vi "Get Target Branch Names.vi"(8 "error in":errorcluster, 11 "Peer Review in":refnum<class "Peer Review.lvclass">) -> (0 "error out":errorcluster, 3 "Peer Review out":refnum<class "Peer Review.lvclass">)   [LabVIEW 2020, in "Peer Review.lvclass"]
uses:
  Peer Review.lvclass
  Peer Review.lvclass/Peer Review.ctl
  <vilib>/Utility/error.llb/Trim Whitespace One-Sided.vi
  <vilib>/regexp/Match Regular Expression.xnode
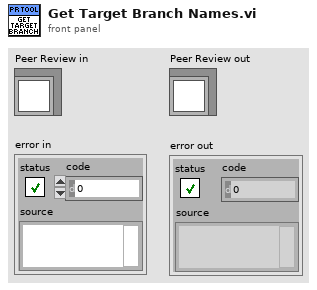
[diagram p1: front panel]
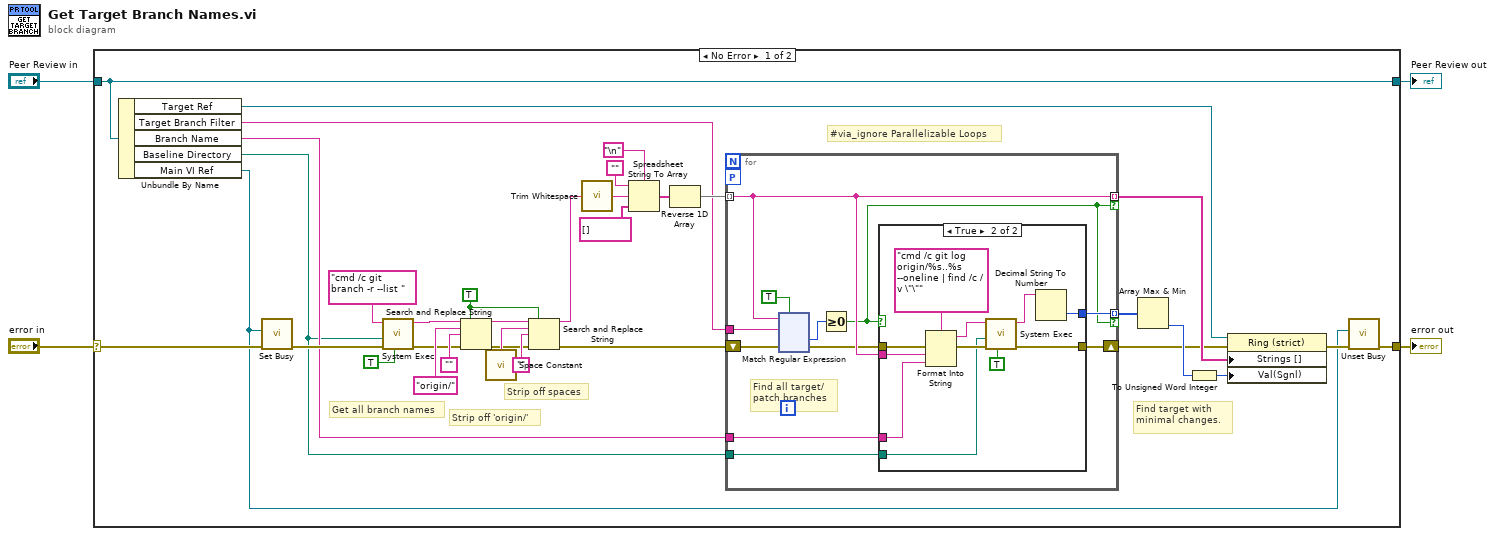
[diagram p0: block diagram]
diagram:
  n1 = case shown="No Error" "error in" {
    selector: "error in" -> [w34 w179]
    tunnel: [w32 w179] -> w3
    tunnel: [w38 w180] -> w4
    tunnel: "Peer Review in" -> [w38 w180]
    frame No Error {
      w14 = TRUE ("replace all? (F)")
      # "#via_ignore Parallelizable Loops"
      # "Find target with minimal changes."
      # "Strip off spaces"
      # "Strip off 'origin/'"
      # "Get all branch names"
      n2 = Unbundle By Name(w38) -> ("Target Ref"=w37:refnum<vi>, "Target Branch Filter"=w5:string, "Branch Name"=w11:string, "Baseline Directory"=w10:path, "Main VI Ref"=w13:refnum<vi>)
      n3 = call <vilib>:"Set Busy.vi"("error in (no error)"=w34, "VI reference (current VI)"=w13) -> ("error out"=w16:errorcluster)  [unwired: 8 in, 1 out]
      n4 = call <vilib>:"System Exec.vi"("run minimized? (F)"=TRUE, "error in (no error)"=w16, "working directory"=w10, "command line"="cmd /c git branch -r --list " ("String 2")) -> ("error out"=w22:errorcluster, "standard output"=w24:string)  [unwired: 4 in, 2 out]
      n5 = Search and Replace String(replace all?=w14, input string=w24, search string="origin/", replace string="" ("Empty String Constant"), error in=w22) -> (result string=w28:string, error out=w25:errorcluster)  [unwired: 3 in, 2 out]
      n6 = call <vilib>:"Space Constant.vi"() -> ("String"=w26:string)
      n7 = Search and Replace String(replace all?=w14, input string=w28, search string=w26, replace string="" ("Empty String Constant"), error in=w25) -> (result string=w7:string, error out=w12:errorcluster)  [unwired: 3 in, 2 out]
      n8 = call <vilib>:"Trim Whitespace.vi"("string"=w7) -> ("trimmed string"=w6:string)  [unwired: 1 in]
      n9 = Spreadsheet String To Array(delimiter (Tab)="\n" ("Line Feed Constant"), format string="", spreadsheet string=w6, array type (2D Dbl)=string[] [] ("Strings []")) -> (array=w18:string[])
      n10 = Reverse 1D Array(array=w18) -> (reversed array=w17:string[])
      n11 = for {
        tunnel: w17 -> [w43] mode=indexing
        tunnel: [w43] -> w15 mode=indexing if=w39
        workers-P: _ -> [_]
        tunnel: w11 -> [w48]
        tunnel: [w47] -> w9 mode=indexing if=w39
        tunnel: w10 -> [w46]
        shift-right: [w49] -> w8
        shift-left: w12 -> [w42]
        tunnel: w5 -> [w44]
        # "Find all target/patch branches"
        n12 = xnode "Match Regular Expression"("input string"=w43, "regular expression"=w44, "error in"=w42, "ignore case? (F)"=TRUE) -> ("offset past match"=w40:i32, "error out"=w41:errorcluster)  [unwired: 2 in, 3 out]
        n13 = Greater Or Equal To 0?(x=w40) -> (x >= 0?=w39:bool)
        n14 = case shown="True" w39 {
          tunnel: w41 -> [w167 w174]
          tunnel: [w167 w173] -> w49
          tunnel: w43 -> [_ w172]
          tunnel: w48 -> [_ w171]
          tunnel: [_ w168] -> w47
          tunnel: w46 -> [_ w169]
          frame False {
          }
          frame True {
            n15 = Format Into String(format string="cmd /c git log origin/%s..%s --oneline | find /c /v \"\"" ("String 2"), error in=w174, w172, w171) -> (resulting string=w177:string, error out=w175:errorcluster)  [unwired: 1 in]
            n16 = call <vilib>:"System Exec.vi"("run minimized? (F)"=TRUE, "error in (no error)"=w175, "working directory"=w169, "command line"=w177) -> ("error out"=w173:errorcluster, "standard output"=w170:string)  [unwired: 4 in, 2 out]
            n17 = Decimal String To Number(string=w170) -> (number=w168:i32)  [unwired: 2 in, 1 out]
          }
        }
      }
      n18 = Array Max & Min(array=w9) -> (min index (indices)=w36:i32)  [unwired: 3 out]
      n19 = To Unsigned Word Integer(number=w36) -> (unsigned 16bit integer=w35:u16)
      n20 = property on="Property Node" class="Ring (strict)"(reference=w37, error in=w8, "Strings []"=w15, "Val(Sgnl)"=w35) -> (error out=w33:errorcluster)  [unwired: 1 out]
      n21 = call <vilib>:"Unset Busy.vi"("error in (no error)"=w33, "VI reference (current VI)"=w13) -> ("error out"=w32:errorcluster)  [unwired: 9 in]
    }
    frame Error {
    }
  }
  "error out" <- w3
  "Peer Review out" <- w4
